vi "Register Collector.vi"(8 "error in (no error)":errorcluster, 10 "Collector":refnum<class "Collectable.lvclass">, 11 "Session Handle in":T1) -> (0 "error out":errorcluster, 3 "Session Handle out":T1)   [LabVIEW 2020, in "Registry.lvlib" / "Registry Session.lvclass"]
uses:
  Registry Session.lvclass
  Typedefs/Session Handle.ctl
  collector/collectable/Collectable.lvclass
  Registry Session.lvclass/Registry Session.ctl
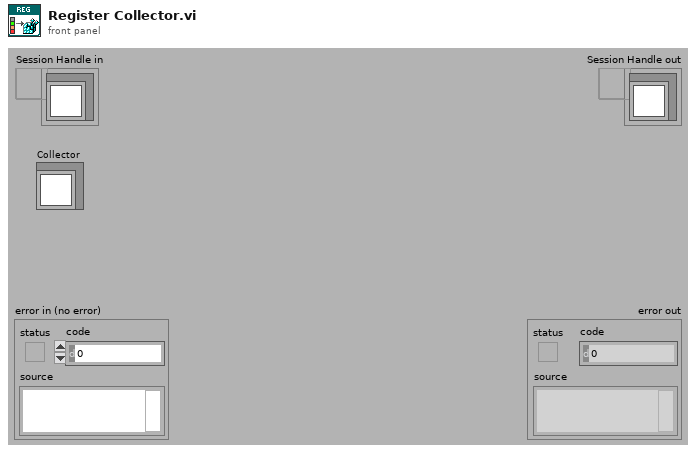
[diagram p1: front panel]
types:
  T1 = typedef "Registry.lvlib/Registry Session.lvclass/Session Handle.ctl" = refnum<data-value>
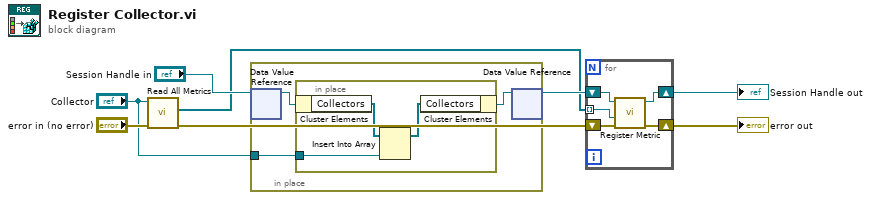
[diagram p0: block diagram]
diagram:
  n1 = call-dynamic "Read All Metrics.vi"("error in (no error)"="error in (no error)", "Collectable in"="Collector") -> ("error out"=w1:errorcluster, "Metrics"=w2:refnum<data-value>[])  [unwired: 7 in, 1 out]
  n2 = in-place {
    in-place-border: "Collector" -> [w10]
    n3 = in-place-dvr #1("Session Handle in") -> (w11:refnum<class "Registry Session.lvclass">)  [unwired: 1 out]
    n4 = in-place {
      in-place-border: w10 -> [w12]
      n5 = in-place-cluster #2(w11) -> ("Collectors"=w14:refnum<class "Collectable.lvclass">[])
      n6 = Insert Into Array(array=w14, new element=w12) -> (w13:refnum<class "Collectable.lvclass">[])  [unwired: 1 in]
      n7 = in-place-cluster #2("Collectors"=w13) -> (w9:refnum<class "Registry Session.lvclass">)
    }
    n8 = in-place-dvr #1(w9) -> (w5:T1)  [unwired: 1 out]
  }
  n9 = for {
    shift-right: [w18] -> w8
    shift-left: w5 -> [w19]
    shift-right: [w15] -> w7
    shift-left: w1 -> [w17]
    tunnel: w2 -> [w16] mode=indexing
    n10 = call "Register Metric.vi"("error in (no error)"=w17, "New Metric"=w16, "Session Handle in"=w19) -> ("error out"=w15:errorcluster, "Session Handle out"=w18:T1)  [unwired: 7 in]
  }
  "Session Handle out" <- w8
  "error out" <- w7
